vi "Game_New.vi"(0 "State":T1={"Tick"=0, "Phase"=0, "PhaseTicks"=0, "Level"=1, "Room"=0, "X10"=0, "Y10"=0, "VY10"=0, "Mode"=0, "Facing"=0, "Run"=0, "Vert"=0, "StandY"=0, "EntryX10"=0, "EntryY10"=0, "EntryMode"=0, "Lives"=4, "Score"=0, "NextLife"=10000, "KeyR"=0, "KeyB"=0, "KeyY"=0, "Torch"=FALSE, "FloorPhase"=0, "Dead"=FALSE, "LevelStart"=FALSE, "Quit"=FALSE, "Sound"=0, "Seed"=12345, "DemoStep"=0, "Tiles"=[], "World"=[], "Enemies"=[], "Highscores"=[], "Name"=[0, 0, 0], "Cursor"=0}, 5 "Rooms":T2(array[cluster]), 7 "Demo":bool, 11 "error in":errorcluster) -> (4 "State out":T1={"Tick"=0, "Phase"=0, "PhaseTicks"=0, "Level"=1, "Room"=0, "X10"=0, "Y10"=0, "VY10"=0, "Mode"=0, "Facing"=0, "Run"=0, "Vert"=0, "StandY"=0, "EntryX10"=0, "EntryY10"=0, "EntryMode"=0, "Lives"=4, "Score"=0, "NextLife"=10000, "KeyR"=0, "KeyB"=0, "KeyY"=0, "Torch"=FALSE, "FloorPhase"=0, "Dead"=FALSE, "LevelStart"=FALSE, "Quit"=FALSE, "Sound"=0, "Seed"=12345, "DemoStep"=0, "Tiles"=[], "World"=[], "Enemies"=[], "Highscores"=[], "Name"=[0, 0, 0], "Cursor"=0}, 15 "error out":errorcluster)   [LabVIEW 2020, in "GH_Engine.lvlib"]
doc: "Starts a new game: 4 lives, score 0, next extra life at 10000, level 1 (Level_Setup). Tick starts at 0 (same rhythm of the vanishing floors every time). Demo: the same game, but in phase Demo with a fixed random seed."
uses:
  GH_Engine.lvlib
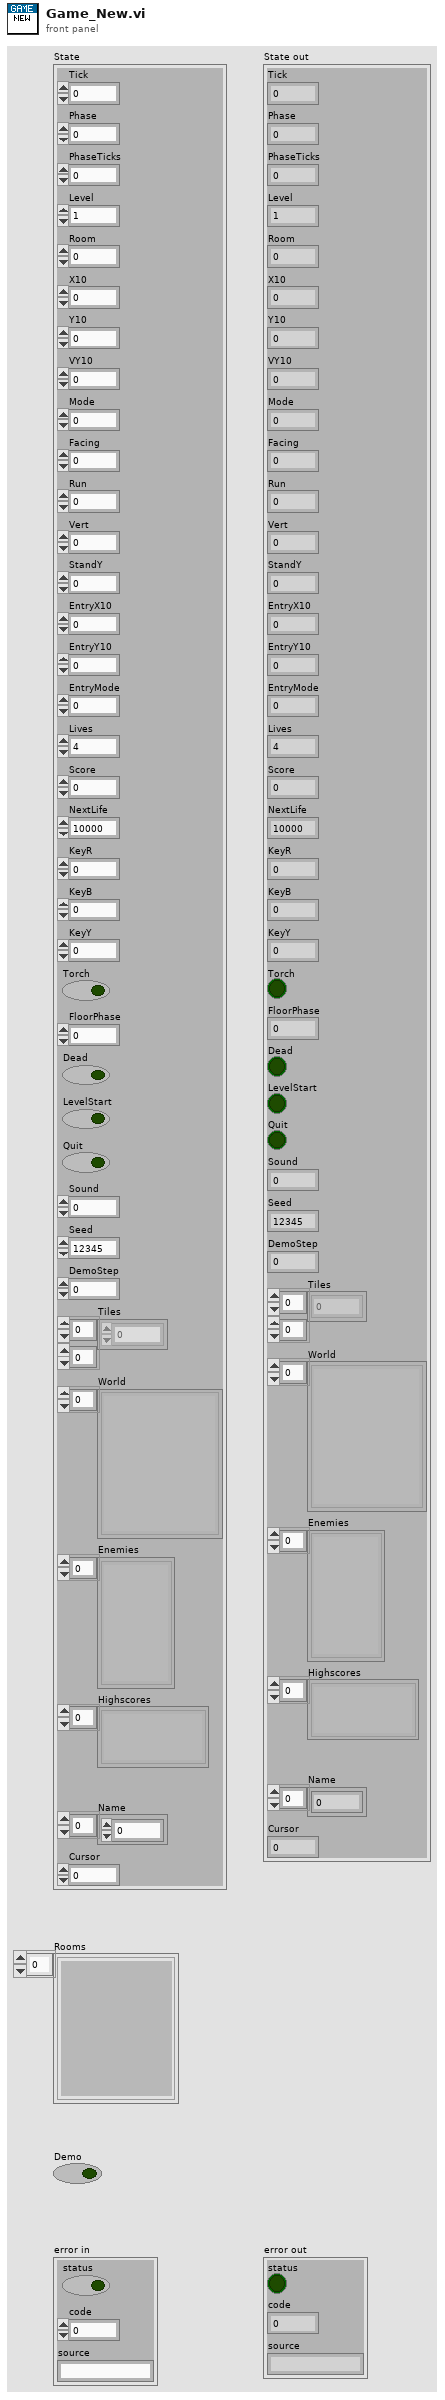
[diagram p1: front panel]
types:
  T1 = cluster{"Tick":u32, "Phase":i32, "PhaseTicks":i32, "Level":i32, "Room":i32, "X10":i32, "Y10":i32, "VY10":i32, "Mode":i32, "Facing":i32, "Run":i32, "Vert":i32, "StandY":i32, "EntryX10":i32, "EntryY10":i32, "EntryMode":i32, "Lives":i32, "Score":i32, "NextLife":i32, "KeyR":i32, "KeyB":i32, "KeyY":i32, "Torch":bool, "FloorPhase":i32, "Dead":bool, "LevelStart":bool, "Quit":bool, "Sound":i32, "Seed":u32, "DemoStep":i32, "Tiles":u8[][], "World":cluster{"ID":string, "Depth":i32, "Column":i32, "Tiles":u8[][]}[], "Enemies":cluster{"Kind":i32, "X10":i32, "Y10":i32, "Dir":i32, "Mode":i32}[], "Highscores":cluster{"Score":i32, "Name":string}[], "Name":i32[], "Cursor":i32}
  T2 = cluster{"ID":string, "Depth":i32, "Column":i32, "Tiles":u8[][]}[]
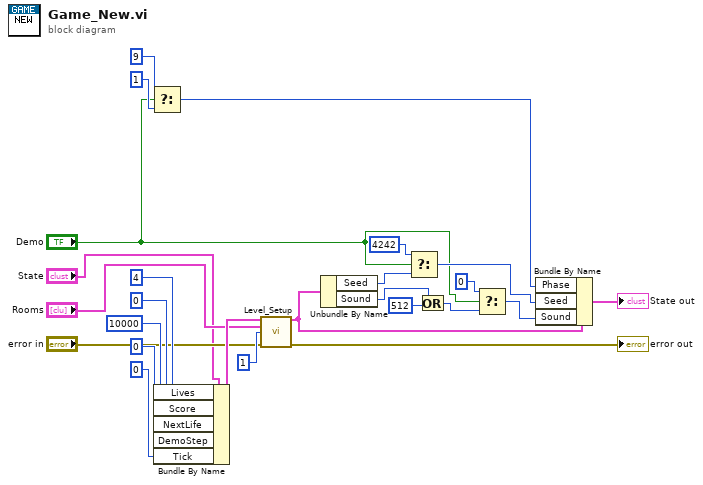
[diagram p0: block diagram]
diagram:
  n1 = Select(t=9, s="Demo", f=1) -> (s? t:f=w18:i32)
  n2 = Bundle By Name(cluster="State", "Lives"=4, "Score"=0, "NextLife"=10000, "DemoStep"=0, "Tick"=u32 0) -> (w10:T1)
  n3 = call "Level_Setup.vi"("State"=w10, "Rooms"="Rooms", "Level"=1, "error in"="error in") -> ("State out"=w12:T1, "error out"=→"error out":errorcluster)  [unwired: 10 in]
  n4 = Unbundle By Name(w12) -> ("Seed"=w14:u32, "Sound"=w15:i32)
  n5 = Select(t=u32 4242, s="Demo", f=w14) -> (s? t:f=w20:u32)
  n6 = Or(x=w15, y=512) -> (x .or. y?=w23:i32)
  n7 = Select(t=0, s="Demo", f=w23) -> (s? t:f=w24:i32)
  n8 = Bundle By Name(cluster=w12, "Phase"=w18, "Seed"=w20, "Sound"=w24) -> (→"State out":T1)
